vi "Panel.vi"(11 "Cloned Panel in":refnum<class "Cloned Panel.lvclass">) -> ()   [LabVIEW 2020, in "Cloned UI.lvlib" / "Cloned Panel.lvclass"]
uses:
  Cloned Panel.lvclass
  OOPanel/Panel/Panel.lvclass
  OOPanel/OOPanel.lvlib
panel:
  out "Iterations":i32
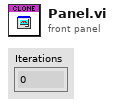
[diagram p1: front panel]
types:
  T1 = enum32{"Invalid", "Standard", "Closed", "Hidden", "Minimized", "Maximized"}
  T2 = typedef "eventsource.ctl" = u32
  T3 = typedef "OOPanel.lvlib/Visibility State.ctl" = enum16{"Idle", "Closed", "Hidden", "Visible", "Subpanel", "Hidden Subpanel"}
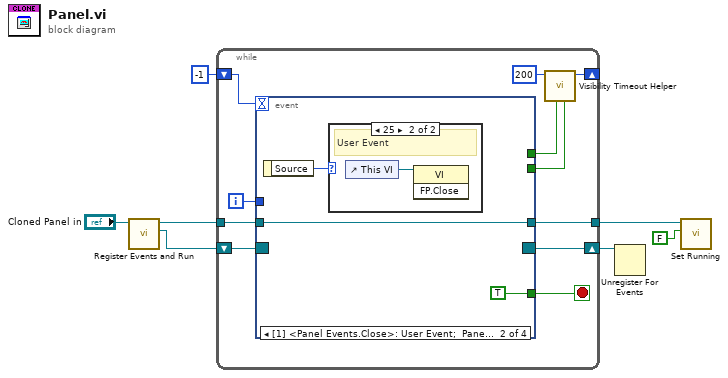
[diagram p0: block diagram]
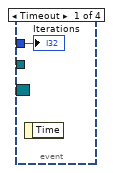
[diagram p2: hidden frame]
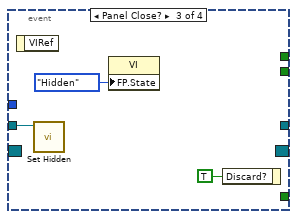
[diagram p4: hidden frame]
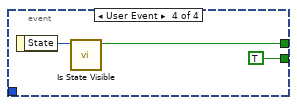
[diagram p5: hidden frame]
diagram:
  n1 = call "Register Events and Run.vi"("Panel in"="Cloned Panel in") -> ("Panel Event Reg"=w5:refnum<event-registration>, "Panel out"=w6:refnum<class "Cloned Panel.lvclass">)  [unwired: 8 in, 1 out]
  n2 = while {
    tunnel: w6 -> [w10]
    shift-right: [w18] -> w1
    shift-left: w5 -> [w8]
    shift-right: [w16] -> _
    shift-left: -1 -> [w15]
    tunnel: [w9] -> w3
    i -> [w12]
    stop <- w11 stop-if-true
    n3 = event shown="[1] <Panel Events.Close>: User Event;  Panel Close" {
      selector: w8 -> [_ _ _ _]
      dyn-events: [_ _ _ _] -> w18
      timeout: w15 -> [_ _ _ _]
      tunnel: [_ _ _ w28] -> w14
      tunnel: [_ _ _ TRUE] -> w13
      tunnel: w12 -> [w19 _ _ _]
      tunnel: [_ TRUE _ _] -> w11
      tunnel: w10 -> [_ w21 w25 _]
      tunnel: [_ w21 _ _] -> w9
      event Timeout {
        n4 = event-data() -> ()  [unwired: 1 in, 1 out]
        "Iterations" <- w19
      }
      event User Event; Panel Close {
        n5 = event-data() -> ("Source"=w20:T2)  [unwired: 1 in]
        n6 = case shown="25" w20 {
          frame Default {
            # "LabVIEW UI"
          }
          frame 25 {
            # "User Event"
            n7 = control-ref of="This VI"() -> (w23:refnum<vi>)
            n8 = invoke class="VI" method="FP.Close"(reference=w23) -> ()  [unwired: 2 in, 3 out]
          }
        }
      }
      event Panel Close? {
        n9 = event-data() -> ()  [unwired: 1 in, 1 out]
        n10 = call "Set Hidden.vi"("Panel in"=w25) -> ()  [unwired: 9 in, 2 out]
        n11 = property class="VI"("FP.State"=T1."Hidden" ("Front Panel Window:State")) -> ()  [unwired: 2 in, 2 out]
        n12 = event-data("Discard?"=TRUE) -> ()  [unwired: 1 in, 1 out]
      }
      event User Event {
        n13 = event-data() -> ("State"=w29:T3)  [unwired: 1 in]
        n14 = call "Is State Visible.vi"("Visibility"=w29) -> ("Visible"=w28:bool)  [unwired: 10 in]
      }
    }
    n15 = call "Visibility Timeout Helper.vi"("Update?"=w13, "Use Timeout?"=w14, "Visible Timeout mS"=200) -> ("Timeout"=w16:i32)  [unwired: 8 in]
  }
  n16 = Unregister For Events(event registration refnum=w1) -> ()  [unwired: 1 in, 1 out]
  n17 = call "Set Running.vi"("Running"=FALSE, "Panel in"=w3) -> ()  [unwired: 8 in, 2 out]
